vi "Add Protection.vi"(8 "error in (no error)":errorcluster, 9 "Pad":bool, 10 "String in":string, 11 "SMC Protection in":refnum<class "SMC Protection.lvclass">) -> (0 "error out":errorcluster, 2 "String out":string, 3 "SMC Protection out":refnum<class "SMC Protection.lvclass">)   [LabVIEW 2026, in "Protections.lvlib" / "SMC Protection.lvclass"]
uses:
  SMC Protection.lvclass
panel:
  # ":011700000002000D000102F64D"
  # ":0117040E350123"
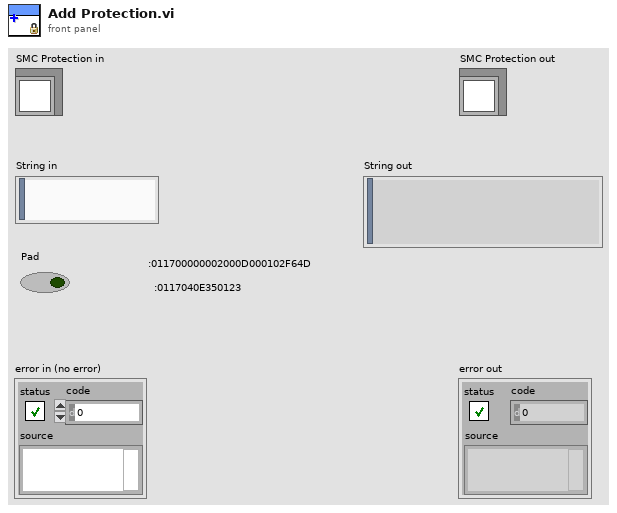
[diagram p1: front panel]
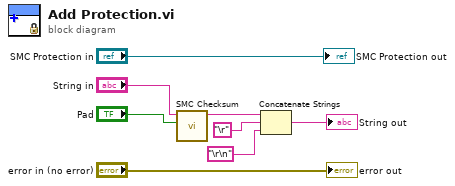
[diagram p0: block diagram]
diagram:
  n1 = call "SMC Checksum.vi"("Pad"="Pad", "String in"="String in") -> ("result string"=w4:string)  [unwired: 8 in, 1 out]
  n2 = Concatenate Strings(w4, "\r", "\r\n") -> (→"String out":string)
  "error out" <- "error in (no error)"
  "SMC Protection out" <- "SMC Protection in"
